vi "Transaction ID Test.vi"() -> ()   [LabVIEW 2012]
uses:
  <vilib>/NI/Modbus Library/Data Model/Device Data Model.lvclass
  MB_ADU_TCP/MB_ADU_TCP.lvclass
  MB_Master_TCP/MB_Master_TCP.lvclass
  MB_ADU_TCP/MB_ADU_TCP.lvclass/MB_ADU_TCP.ctl
  <vilib>/NI/Modbus Library/API/Slave/Modbus Slave.lvclass
  MB_ADU_TCP/Read Transaction ID.vi
  <vilib>/NI/Modbus Library/API/Wrapper/Create TCP Slave.vi
  MB_ADU/MB_ADU.lvclass
  <vilib>/NI/Modbus Library/API/Wrapper/API Main.lvlib
  MB Master.lvlib
panel:
  out "Slave coil":bool
  out "Transaction ID 3":u16
  in  "stop 3":bool
  out "Coils 3":bool[](array[boolean])
  out "Coils 2":bool[](array[boolean])
  out "Coils 1":bool[](array[boolean])
  out "Transaction ID 2":u16
  in  "stop 2":bool
  in  "stop 1":bool
  out "Transaction ID 1":u16
  in  "stop slave":bool
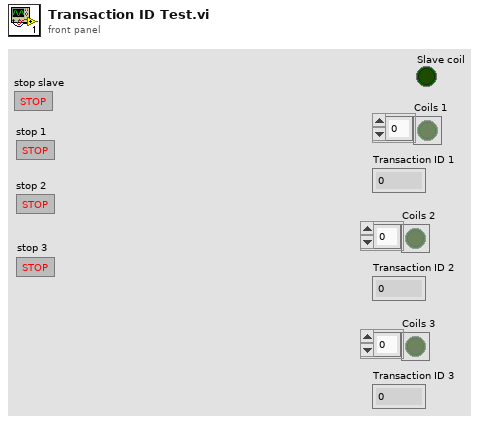
[diagram p1: front panel]
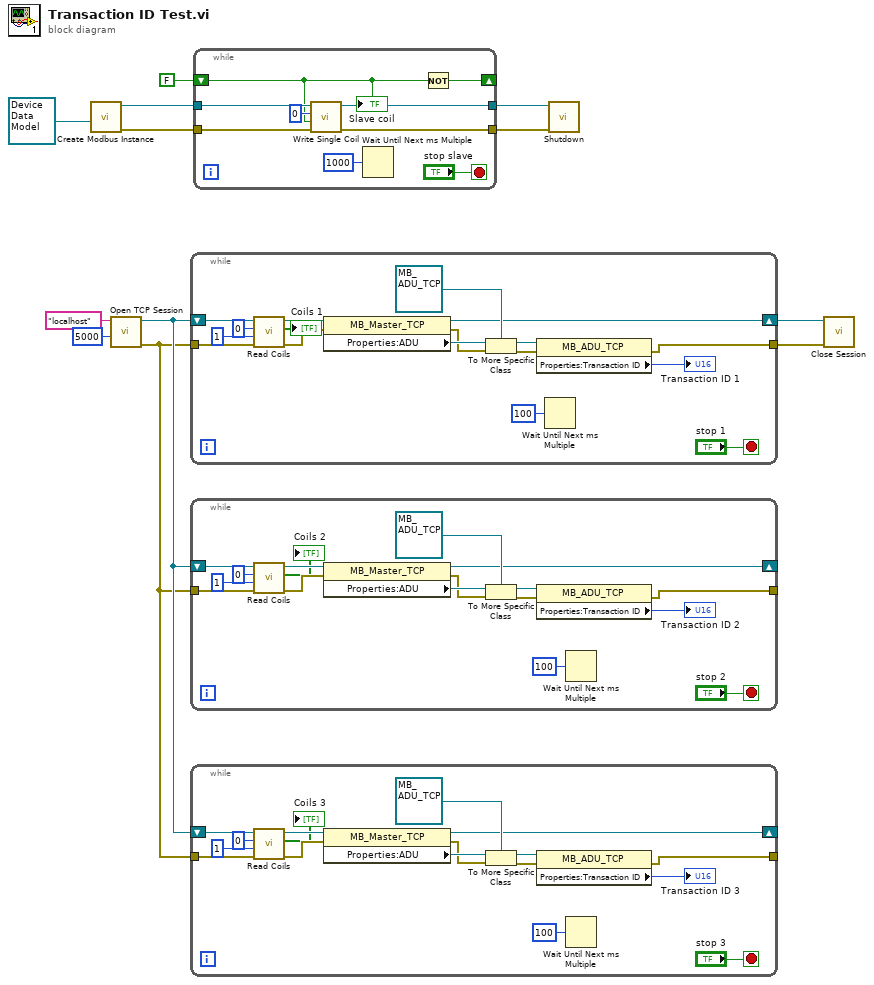
[diagram p0: block diagram]
diagram:
  n1 = call-poly <vilib>:"Create Modbus Instance.vi"("device data model"=refnum<class "Device Data Model.lvclass"> refnum) -> ("error out"=w10:errorcluster, "TCP slave instance"=w11:refnum<class "Modbus Slave.lvclass">)  [unwired: 9 in]
  n2 = call "Open TCP Session.vi"("Timeout (10000)"=5000, "IP Address"="localhost") -> ("error out"=w1:errorcluster, "MB_TCP session"=w2:refnum<class "MB_Master_TCP.lvclass">)  [unwired: 8 in]
  n3 = while {
    tunnel: w1 -> [w28]
    shift-right: [w17] -> w4
    shift-left: w2 -> [w29]
    tunnel: [w15] -> w3
    stop <- "stop 1" stop-if-true
    n4 = call "Read Coils.vi"("error in (no error)"=w28, "quantity"=u16 1, "starting address"=u16 0, "MB session in"=w29) -> ("error out"=w24:errorcluster, "Coils"=→"Coils 1":bool[], "MB session out"=w25:refnum<class "MB_Master_TCP.lvclass">)  [unwired: 5 in]
    n5 = property class="MB_Master_TCP"(reference=w25, error in=w24) -> (reference out=w17:refnum<class "MB_Master_TCP.lvclass">, error out=w22:errorcluster, "Properties:ADU"=w23:refnum<class "MB_ADU.lvclass">)
    n6 = To More Specific Class(target class=refnum<class "MB_ADU_TCP.lvclass"> refnum ("MB Serial Master:MB_ADU_TCP"), reference=w23, error in=w22) -> (specific class reference=w20:refnum<class "MB_ADU_TCP.lvclass">, error out=w19:errorcluster)
    n7 = property class="MB_ADU_TCP"(reference=w20, error in=w19) -> (error out=w15:errorcluster, "Properties:Transaction ID"=→"Transaction ID 1":u16)  [unwired: 1 out]
    n8 = Wait Until Next ms Multiple(millisecond multiple=u32 100) -> ()  [unwired: 1 out]
  }
  n9 = while {
    tunnel: w1 -> [w45]
    shift-right: [w34] -> _
    shift-left: w2 -> [w46]
    tunnel: [w32] -> _
    stop <- "stop 2" stop-if-true
    n10 = call "Read Coils.vi"("error in (no error)"=w45, "quantity"=u16 1, "starting address"=u16 0, "MB session in"=w46) -> ("error out"=w41:errorcluster, "Coils"=→"Coils 2":bool[], "MB session out"=w42:refnum<class "MB_Master_TCP.lvclass">)  [unwired: 5 in]
    n11 = property class="MB_Master_TCP"(reference=w42, error in=w41) -> (reference out=w34:refnum<class "MB_Master_TCP.lvclass">, error out=w39:errorcluster, "Properties:ADU"=w40:refnum<class "MB_ADU.lvclass">)
    n12 = To More Specific Class(target class=refnum<class "MB_ADU_TCP.lvclass"> refnum ("MB Serial Master:MB_ADU_TCP"), reference=w40, error in=w39) -> (specific class reference=w37:refnum<class "MB_ADU_TCP.lvclass">, error out=w36:errorcluster)
    n13 = property class="MB_ADU_TCP"(reference=w37, error in=w36) -> (error out=w32:errorcluster, "Properties:Transaction ID"=→"Transaction ID 2":u16)  [unwired: 1 out]
    n14 = Wait Until Next ms Multiple(millisecond multiple=u32 100) -> ()  [unwired: 1 out]
  }
  n15 = while {
    tunnel: w1 -> [w62]
    shift-right: [w51] -> _
    shift-left: w2 -> [w63]
    tunnel: [w49] -> _
    stop <- "stop 3" stop-if-true
    n16 = call "Read Coils.vi"("error in (no error)"=w62, "quantity"=u16 1, "starting address"=u16 0, "MB session in"=w63) -> ("error out"=w58:errorcluster, "Coils"=→"Coils 3":bool[], "MB session out"=w59:refnum<class "MB_Master_TCP.lvclass">)  [unwired: 5 in]
    n17 = property class="MB_Master_TCP"(reference=w59, error in=w58) -> (reference out=w51:refnum<class "MB_Master_TCP.lvclass">, error out=w56:errorcluster, "Properties:ADU"=w57:refnum<class "MB_ADU.lvclass">)
    n18 = To More Specific Class(target class=refnum<class "MB_ADU_TCP.lvclass"> refnum ("MB Serial Master:MB_ADU_TCP"), reference=w57, error in=w56) -> (specific class reference=w54:refnum<class "MB_ADU_TCP.lvclass">, error out=w53:errorcluster)
    n19 = property class="MB_ADU_TCP"(reference=w54, error in=w53) -> (error out=w49:errorcluster, "Properties:Transaction ID"=→"Transaction ID 3":u16)  [unwired: 1 out]
    n20 = Wait Until Next ms Multiple(millisecond multiple=u32 100) -> ()  [unwired: 1 out]
  }
  n21 = while {
    tunnel: w11 -> [w72]
    tunnel: w10 -> [w71]
    tunnel: [w69] -> w9
    tunnel: [w68] -> w8
    shift-right: [w66] -> _
    shift-left: FALSE -> [w65]
    stop <- "stop slave" stop-if-true
    n22 = call-dynamic "Write Single Coil.vi"("error in"=w71, "coil to write"=w65, "address"=u16 0, "Modbus slave in"=w72) -> ("error out"=w68:errorcluster, "Modbus slave out"=w69:refnum<class "Modbus Slave.lvclass">)  [unwired: 6 in]
    n23 = Wait Until Next ms Multiple(millisecond multiple=u32 1000) -> ()  [unwired: 1 out]
    n24 = Not(x=w65) -> (.not. x?=w66:bool)
    "Slave coil" <- w65
  }
  n25 = call-dynamic "Shutdown.vi"("error in"=w8, "Modbus slave in"=w9) -> ()  [unwired: 9 in, 1 out]
  n26 = call-dynamic "Close Session.vi"("error in (no error)"=w3, "MB TCP session"=w4) -> ()  [unwired: 9 in, 1 out]
